vi "Assert Wrapper.vi"(4 "Execution time (s)":dbl=-1.0, 5 "Assert Only? (F)":bool, 6 "error code (1)":i32=1, 7 "Label":string, 8 "error in (no error)":errorcluster, 9 "Register with caller test (F)":bool, 11 "Assert?":bool) -> (0 "error out":errorcluster, 1 "Verbose":bool, 2 "Properties.Assert":refnum<class "Properties.Assert.lvclass">, 3 "Assert out":refnum<class "Assert.lvclass">)   [LabVIEW 2013, in "Caraya.lvlib" / "Assert.lvclass"]
uses:
  Assert.lvclass
  Properties.Assert/Properties.Assert.lvclass
  Test Assert Factory/Test Assert Factory.lvclass
  Assert.lvclass/Assert.ctl
  Assert Factory Manager/Assert Factory Manager.lvclass
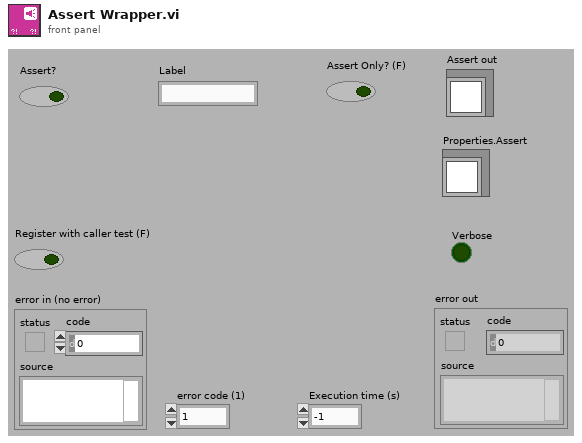
[diagram p1: front panel]
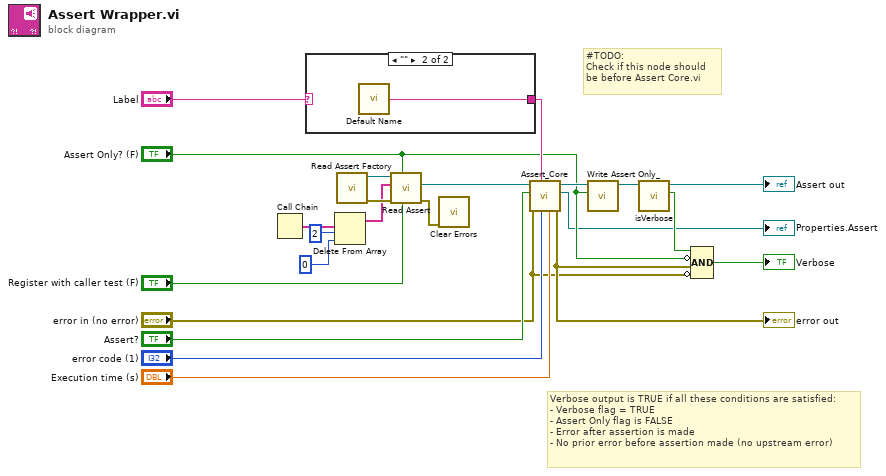
[diagram p0: block diagram]
diagram:
  # "#TODO: \nCheck if this node should\nbe before Assert Core.vi"
  # "Verbose output is TRUE if all these conditions are satisfied: \n- Verbose flag = TRUE\n- Assert Only flag is FALSE\n- Error after assertion is made\n- No prior error before assertion made (no upstream error)"
  n1 = Call Chain() -> (call chain=w5:string[])
  n2 = case shown="\"\"" "Label" {
    selector: "Label" -> [w24 _]
    tunnel: [w24 w25] -> w16
    frame Default {
    }
    frame "" {
      n3 = call "Default Name.vi"() -> ("String"=w25:string)
    }
  }
  n4 = Delete From Array(array=w5, length=2 ("y"), index=0) -> (array with subset deleted=w4:string[])  [unwired: 1 out]
  n5 = call "Read Assert Factory.vi"() -> ("error out"=w19:errorcluster, "Test Assert Factory"=w21:refnum<class "Test Assert Factory.lvclass">)  [unwired: 10 in]
  n6 = call-dynamic "Read Assert.vi"("Register with caller test (F)"="Register with caller test (F)", "Assert Only? (F)"="Assert Only? (F)", "error in (no error)"=w19, "VI Call Chain"=w4, "Assert Factory in"=w21) -> ("error out"=w18:errorcluster, "Assert"=w20:refnum<class "Assert.lvclass">)  [unwired: 4 in, 1 out]
  n7 = call <vilib>:"Clear Errors.vi"("error in (no error)"=w18) -> ()  [unwired: 6 in, 1 out]
  n8 = call "Assert_Core.vi"("Execution time (s)"="Execution time (s)", "error code (1)"="error code (1)", "Name"=w16, "upstream error"="error in (no error)", "Assert?"="Assert?", "Assert in"=w20) -> ("error out"=w8:errorcluster, "Properties.Assert"=→"Properties.Assert":refnum<class "Properties.Assert.lvclass">, "Assert out"=w13:refnum<class "Assert.lvclass">)  [unwired: 3 in]
  "error out" <- w8
  n9 = call "Write Assert Only_.vi"("Assert Only?"="Assert Only? (F)", "Assert"=w13) -> ("Assert"=w11:refnum<class "Assert.lvclass">)  [unwired: 8 in, 1 out]
  n10 = call "isVerbose.vi"("Assert in"=w11) -> ("Verbose"=w12:bool, "Assert out"=→"Assert out":refnum<class "Assert.lvclass">)  [unwired: 9 in]
  n11 = Compound Arithmetic op=AND(w12, invert "Assert Only? (F)", w8, invert "error in (no error)") -> (→"Verbose":bool)
